vi "ZM-PC-getDestinationName.vi"(8 "error in (no error)":errorcluster, 11 "ZM-PC-package in":refnum<class "ZM-PC-package.lvclass">) -> (0 "error out":errorcluster, 2 "destination_name":string, 3 "ZM-PC-package out":refnum<class "ZM-PC-package.lvclass">)   [LabVIEW 2020, in "ZM-PC-packages.lvlib" / "ZM-PC-package.lvclass"]
doc: "Returns the name of the package destination, i.e. the item name of the ZM-PC-DESTINATION enum read through Read destination (Unknown, Root, Hardware or Communication)."
uses:
  ZM-PC-package.lvclass
  ZM-PC-package.lvclass/ZM-PC-package.ctl
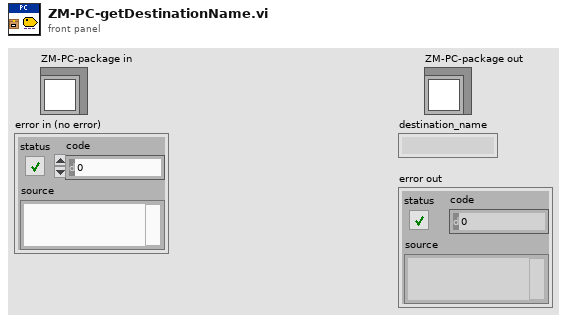
[diagram p1: front panel]
types:
  T1 = typedef "ZM-PC-packages.lvlib/ZM-PC-package.lvclass/ZM-PC-DESTINATION.ctl" = enum16{"Unknown", "Root", "Hardware", "Communication"}
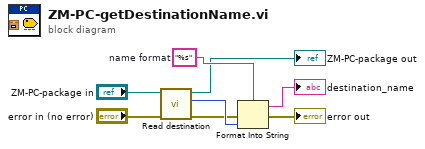
[diagram p0: block diagram]
diagram:
  w6 = "%s"  # name format
  n1 = call "Read destination.vi"("error in (no error)"="error in (no error)", "ZM-PC-package in"="ZM-PC-package in") -> ("error out"=w4:errorcluster, "ZM-PC-DESTINATION"=w5:T1, "ZM-PC-package out"=→"ZM-PC-package out":refnum<class "ZM-PC-package.lvclass">)  [unwired: 7 in]
  n2 = Format Into String(format string=w6, error in=w4, w5) -> (resulting string=→"destination_name":string, error out=→"error out":errorcluster)  [unwired: 1 in]
